vi "Lookup EStop Source.vi"(8 "error in (no error)":errorcluster, 10 "Source Type":string) -> (0 "error out":errorcluster, 3 "Source":refnum<class "EStop Source.lvclass">)   [LabVIEW 2025, in "VolatusControl.lvlib" / "EStop Module.lvclass"]
uses:
  EStop Module.lvclass
  EStop Module.lvclass/EStop Module.ctl
  EStop Source/EStop Source.lvclass
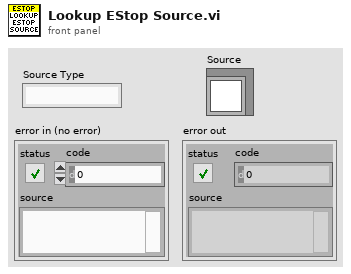
[diagram p1: front panel]
types:
  T1 = map{string, refnum<class "EStop Source.lvclass">}
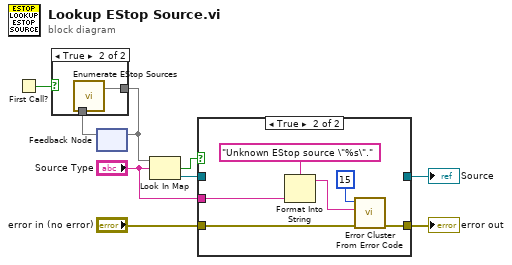
[diagram p0: block diagram]
diagram:
  n1 = First Call?() -> (First Call?: T/F=w9:bool)
  n2 = feedback #1() -> (w8:T1)  [unwired: 1 in]
  n3 = case shown="True" w9 {
    tunnel: [w10 w11] -> w7
    tunnel: w8 -> [w10 _]
    frame False {
    }
    frame True {
      n4 = call "Enumerate EStop Sources.vi"() -> ("Implementation Map"=w11:T1)  [unwired: 7 in]
    }
  }
  n5 = feedback-in #1(w7) -> ()
  n6 = Look In Map(map=w7, key="Source Type") -> (key not found?=w6:bool, value=w5:refnum<class "EStop Source.lvclass">)  [unwired: 1 in]
  n7 = case shown="True" w6 {
    tunnel: w5 -> [w12 _]
    tunnel: "Source Type" -> [_ w17]
    tunnel: [w13 w15] -> w2
    tunnel: "error in (no error)" -> [w13 w14]
    tunnel: [w12 _] -> w1
    frame False {
    }
    frame True {
      n8 = Format Into String(format string="Unknown EStop source \"%s\".", w17) -> (resulting string=w16:string)  [unwired: 2 in, 1 out]
      n9 = call <vilib>:"Error Cluster From Error Code.vi"("error in (no error)"=w14, "error message (\"\")"=w16, "error code (0)"=15) -> ("error out"=w15:errorcluster)  [unwired: 6 in]
    }
  }
  "error out" <- w2
  "Source" <- w1
